vi "selected path_list.vi"(8 "selection":enum16{"10k", "100k"}(ring), 11 "F_array_Link":path[](array[path])) -> (3 "Selected F_array_Link":path[](array[path]))   [LabVIEW 2018]
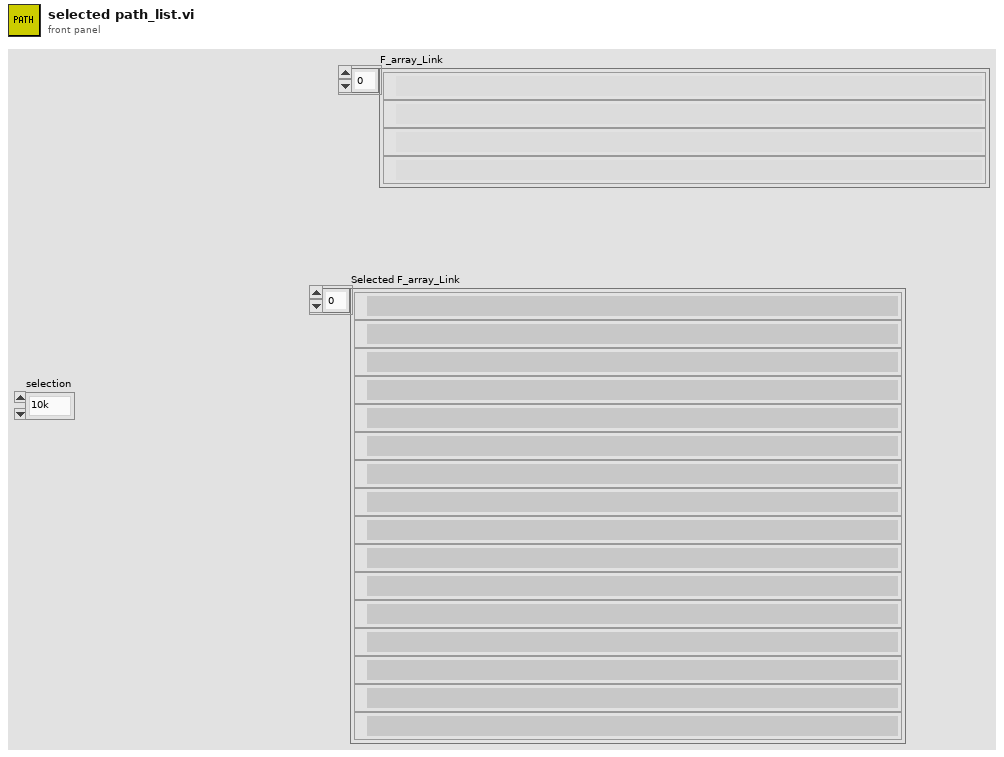
[diagram p1: front panel]
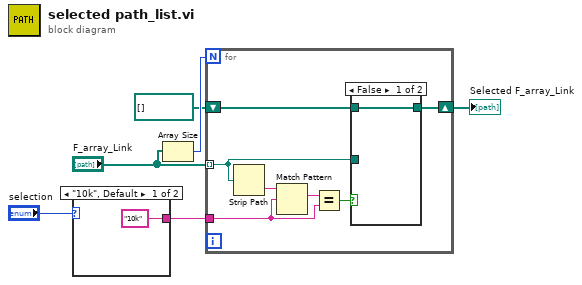
[diagram p0: block diagram]
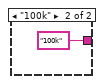
[diagram p2: hidden frame]
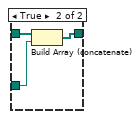
[diagram p3: hidden frame]
diagram:
  n1 = case shown="\"10k\", Default" "selection" {
    tunnel: ["10k" ("search string") "100k" ("search string")] -> w3
    frame "10k", Default {
    }
    frame "100k" {
    }
  }
  n2 = Array Size(array="F_array_Link") -> (size(s)=w6:i32)
  n3 = for {
    N: w6 -> [_]
    tunnel: "F_array_Link" -> [w9] mode=indexing
    tunnel: w3 -> [w12]
    shift-right: [w11] -> w1
    shift-left: path[] [] -> [w10]
    n4 = Strip Path(path=w9) -> (name=w13:string)  [unwired: 1 out]
    n5 = Match Pattern(string=w13, regular expression=w12) -> (match substring=w15:string)  [unwired: 1 in, 3 out]
    n6 = Equal?(x=w15, y=w12) -> (x = y?=w14:bool)
    n7 = case shown="False" w14 {
      tunnel: w9 -> [_ w19]
      tunnel: [w16 w18] -> w11
      tunnel: w10 -> [w16 w17]
      frame False {
      }
      frame True {
        n8 = Build Array (concatenate)(w17, w19) -> (w18:path[])
      }
    }
  }
  "Selected F_array_Link" <- w1
